vi "Serial Port.vi"() -> ()   [LabVIEW 2024]
panel:
  in  "Combo Box":string(combo)
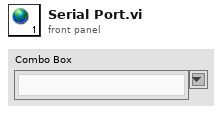
[diagram p1: front panel]
diagram:
